vi "Main.vi"() -> ()   [LabVIEW 2020, in "2D Array Example.lvlib"]
uses:
  2D Array Example.lvlib
  2DArrayPanel/2DArrayPanel.lvclass
  OOPanel/2DArrayManager/2DArrayManager.lvclass
  OOPanel/2D Index.ctl
  OOPanel/OOPanel.lvlib
  2DArrayPanel2/2DArrayPanel2.lvclass
  ExBlank/ExBlank.lvclass
panel:
  out "error out":errorcluster
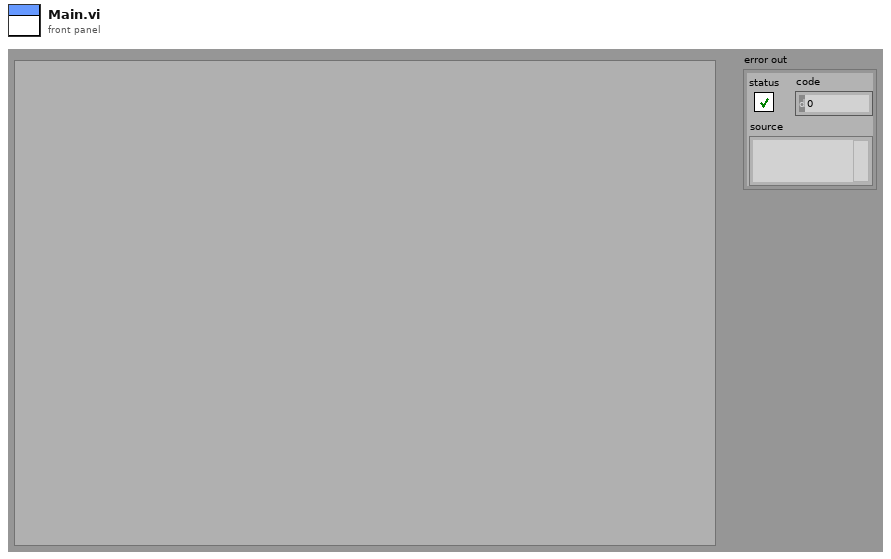
[diagram p1: front panel]
types:
  T1 = typedef "OOPanel.lvlib/2D Index.ctl" = cluster{"Row":i32, "Col":i32}
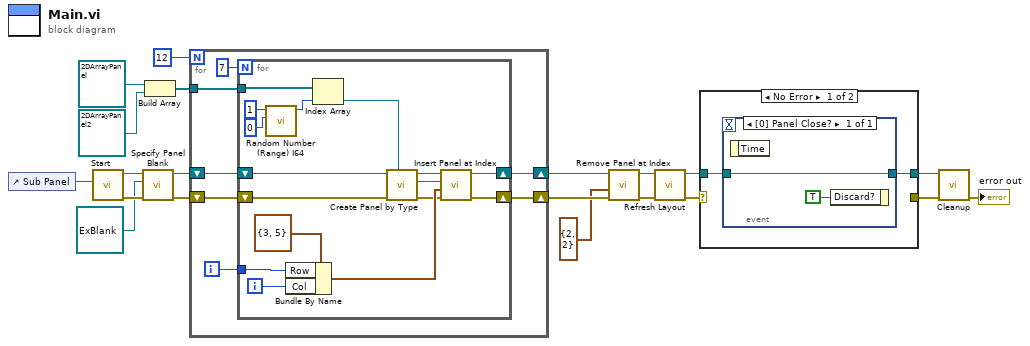
[diagram p0: block diagram]
diagram:
  n1 = control-ref of="Sub Panel"() -> (w19:refnum<vi>)
  n2 = call "Start.vi"("Container"=w19) -> ("error out"=w18:errorcluster, "2DArrayManager out"=w3:refnum<class "2DArrayManager.lvclass">)  [unwired: 9 in]
  n3 = call "Specify Panel Blank.vi"("error in (no error)"=w18, "Blank VI"=refnum<class "ExBlank.lvclass"> refnum ("2D Array Example.lvlib:ExBlank.lvclass"), "2DArrayManager in"=w3) -> ("error out"=w4:errorcluster, "2DArrayManager out"=w2:refnum<class "2DArrayManager.lvclass">)  [unwired: 7 in]
  n4 = Build Array(refnum<class "2DArrayPanel.lvclass"> refnum ("2D Array Example.lvlib:2DArrayPanel.lvclass"), refnum<class "2DArrayPanel2.lvclass"> refnum ("2D Array Example.lvlib:2DArrayPanel2.lvclass")) -> (w6:refnum<class "ArrayPanel.lvclass">[])
  n5 = for {
    N: 12 -> [_]
    shift-right: [w24] -> w10
    shift-left: w2 -> [w26]
    shift-right: [w22] -> w17
    shift-left: w4 -> [w23]
    tunnel: w6 -> [w21]
    i -> [w25]
    n6 = for {
      N: 7 -> [_]
      tunnel: w25 -> [w37]
      shift-right: [w36] -> w24
      shift-left: w26 -> [w43]
      shift-right: [w33] -> w22
      shift-left: w23 -> [w35]
      tunnel: w21 -> [w30]
      i -> [w38]
      n7 = call <vilib>:"Random Number (Range) I64.vi"("lower bound (-100)"=i64 0 ("upper bound (100)"), "upper bound (100)"=i64 1) -> ("number"=w29:i64)  [unwired: 9 in]
      n8 = Bundle By Name(cluster=T1 {"Row"=3, "Col"=5} ("2D Index"), "Row"=w37, "Col"=w38) -> (w39:T1)
      n9 = Index Array(array=w30, index=w29) -> (element=w28:refnum<class "ArrayPanel.lvclass">)
      n10 = call "Create Panel by Type.vi"("Panel Type"=w28, "error in (no error)"=w35, "2DArrayManager in"=w43) -> ("error out"=w34:errorcluster, "Panel"=w41:refnum<class "ArrayPanel.lvclass">, "2DArrayManager out"=w42:refnum<class "2DArrayManager.lvclass">)  [unwired: 6 in]
      n11 = call "Insert Panel at Index.vi"("error in (no error)"=w34, "2D Index"=w39, "ArrayPanel"=w41, "2DArrayManager in"=w42) -> ("error out"=w33:errorcluster, "2DArrayManager out"=w36:refnum<class "2DArrayManager.lvclass">)  [unwired: 4 in, 2 out]
    }
  }
  n12 = call "Remove Panel at Index.vi"("error in (no error)"=w17, "2D Index"=T1 {"Row"=2, "Col"=2}, "2DArrayManager in"=w10) -> ("error out"=w11:errorcluster, "2DArrayManager out"=w9:refnum<class "2DArrayManager.lvclass">)  [unwired: 5 in, 2 out]
  n13 = call "Refresh Layout.vi"("error in (no error)"=w11, "2DArrayManager in"=w9) -> ("error out"=w14:errorcluster, "2DArrayManager out"=w15:refnum<class "2DArrayManager.lvclass">)  [unwired: 8 in]
  n14 = case shown="No Error" w14 {
    selector: w14 -> [_ w48]
    tunnel: [w45 w49] -> w16
    tunnel: w15 -> [w44 w49]
    tunnel: [_ w48] -> w13
    frame No Error {
      n15 = event shown="[0] Panel Close?" {
        selector: _ -> [_]
        dyn-events: _ -> [_]
        timeout: _ -> [_]
        tunnel: [w46] -> w45
        tunnel: w44 -> [w46]
        event Panel Close? {
          n16 = event-data() -> ()  [unwired: 1 in, 1 out]
          n17 = event-data("Discard?"=TRUE) -> ()  [unwired: 1 in, 1 out]
        }
      }
    }
    frame Error {
    }
  }
  n18 = call "Cleanup.vi"("error in (no error)"=w13, "2DArrayManager in"=w16) -> ("error out"=→"error out":errorcluster)  [unwired: 9 in]
